vi "Open CSM_Tool_Launcher.vi"() -> ()   [LabVIEW 2017, in "csm_tool_menu.lvlib"]
uses:
  csm_tool_menu.lvlib
  user.lib/_NEVSTOP/Communicable State Machine(CSM)/_xnode/csm_tool/_xnode_csm_tool_support/CSM DebugTool Dialog.lvlib
  user.lib/_NEVSTOP/Communicable State Machine(CSM)/_tool/_ui/csm-ui-support.lvlib
panel:
  in  "error in (no error)":errorcluster
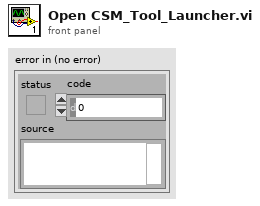
[diagram p1: front panel]
types:
  T1 = enum32{"Invalid", "Standard", "Closed", "Hidden", "Minimized", "Maximized"}
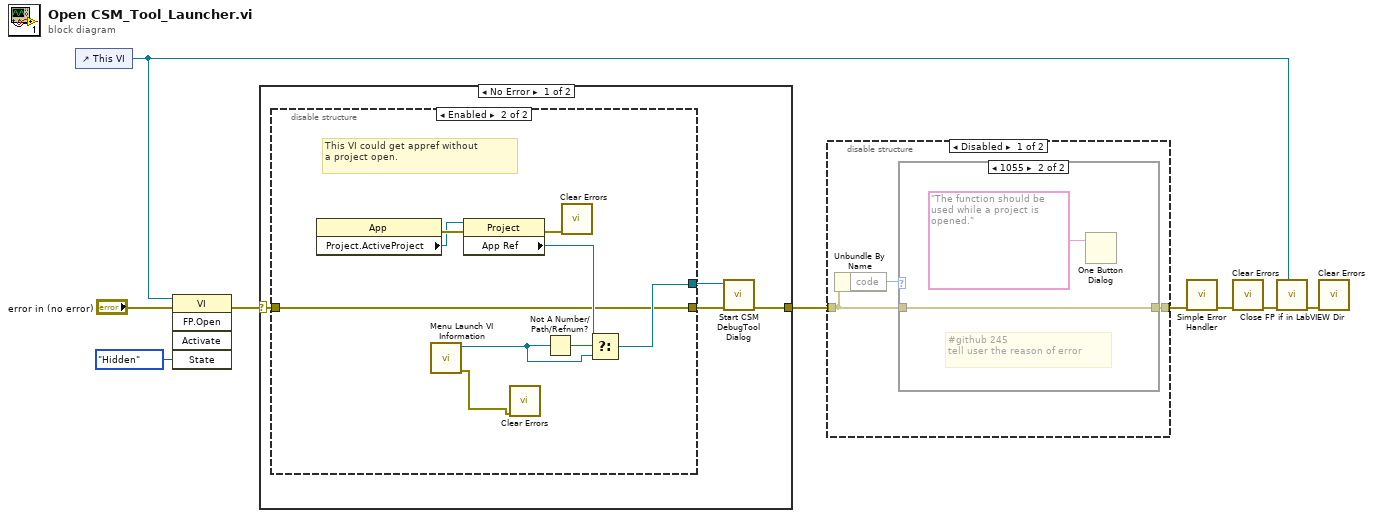
[diagram p0: block diagram]
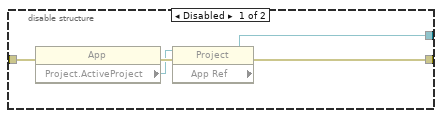
[diagram p2: hidden frame]
diagram:
  n1 = control-ref of="This VI"() -> (w4:refnum<vi>)
  n2 = invoke class="VI" method="FP.Open"(reference=w4, error in="error in (no error)", "State"=T1."Hidden") -> (error out=w5:errorcluster)  [unwired: 2 in, 4 out]
  n3 = case shown="No Error" w5 {
    selector: w5 -> [w13 w28]
    tunnel: [w10 w28] -> w2
    frame No Error {
      n4 = disable-structure shown="Enabled" {
        disable-tunnel: w13 -> [w18 w21]
        disable-tunnel: [w15 w21] -> w12
        disable-tunnel: [w14 w22] -> w11
        frame Disabled {
          n5 = property class="App"(error in=w18) -> (error out=w17:errorcluster, "Project.ActiveProject"=w16:refnum<vi>)  [unwired: 1 in, 1 out]
          n6 = property class="Project"(reference=w16, error in=w17) -> (error out=w15:errorcluster, "App Ref"=w14:refnum<vi>)  [unwired: 1 out]
        }
        frame Enabled {
          # "This VI could get appref without \na project open."
          n7 = property class="App"() -> (error out=w26:errorcluster, "Project.ActiveProject"=w25:refnum<vi>)  [unwired: 2 in, 1 out]
          n8 = call <vilib>:"Menu Launch VI Information.vi"() -> ("error out"=w19:errorcluster, "Menu Launch:App"=w24:refnum<vi>)  [unwired: 9 in, 1 out]
          n9 = property class="Project"(reference=w25, error in=w26) -> (error out=w20:errorcluster, "App Ref"=w23:refnum<vi>)  [unwired: 1 out]
          n10 = call <vilib>:"Clear Errors.vi"("error in (no error)"=w19) -> ()  [unwired: 5 in, 2 out]
          n11 = Not A Number/Path/Refnum?(number/path/refnum=w24) -> (NaN/Path/Refnum?=w27:bool)
          n12 = call <vilib>:"Clear Errors.vi"("error in (no error)"=w20) -> ()  [unwired: 5 in, 2 out]
          n13 = Select(t=w23, s=w27, f=w24) -> (s? t:f=w22:refnum<vi>)
        }
      }
      n14 = call "Start CSM DebugTool Dialog.vi"("error in (no error)"=w12, "Application In"=w11) -> ("error out"=w10:errorcluster)  [unwired: 9 in]
    }
    frame Error {
    }
  }
  n15 = disable-structure shown="Disabled" {
    disable-tunnel: [w31 w35] -> w3
    disable-tunnel: w2 -> [w30 w35]
    frame Disabled {
      n16 = Unbundle By Name(w30) -> ("code"=w29:i32)
      n17 = case shown="1055" w29 {
        tunnel: w30 -> [w32 w34]
        tunnel: [w32 w34] -> w31
        frame 0, Default {
        }
        frame 1055 {
          # "#github 245\ntell user the reason of error"
          n18 = One Button Dialog(message="The function should be used while a project is opened.") -> ()  [unwired: 1 in, 1 out]
        }
      }
    }
    frame Enabled {
    }
  }
  n19 = call <vilib>:"Simple Error Handler.vi"("error in (no error)"=w3) -> ("error out"=w1:errorcluster)  [unwired: 4 in, 4 out]
  n20 = call <vilib>:"Clear Errors.vi"("error in (no error)"=w1) -> ("error out"=w8:errorcluster)  [unwired: 5 in, 1 out]
  n21 = call "Close FP if in LabVIEW Dir.vi"("VI Refnum"=w4, "Error in"=w8) -> ("Error out"=w9:errorcluster)  [unwired: 9 in]
  n22 = call <vilib>:"Clear Errors.vi"("error in (no error)"=w9) -> ()  [unwired: 5 in, 2 out]
